vi "PathPlanner_Cmd_Follow_Internal_InitEvents.vi"(8 "TrigerEvents":bool, 9 "Reset In":bool, 11 "TrajectoryEventCommands":T5) -> (3 "UntriggeredEvents":T1[](array[typedef]))   [LabVIEW 2019, in "PathPlanner24.lvlib"]
doc: "This is an internal function. It is not to be called by end users."
uses:
  PathPlanner24.lvlib
  ENum/PathPlanner_TrajectoryEvent_Type_ENUM.ctl
  TypeDef/PathPlannerCommandUtil.ctl
  TypeDef/PathPlannerTrajectoryEvent.ctl
  ENum/PathPlanner_CommandUtil_Type_ENUM.ctl
  TypeDef/PathPlannerTrajectoryEvents.ctl
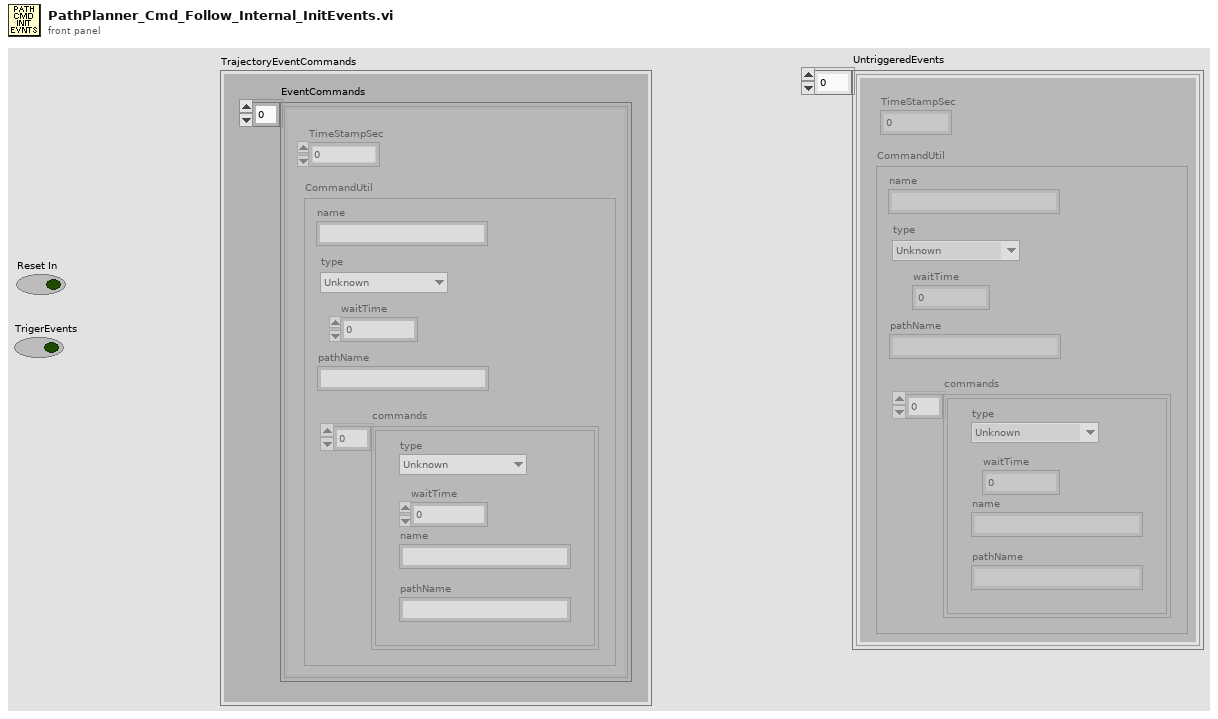
[diagram p1: front panel]
types:
  T1 = typedef "PathPlanner24.lvlib/PathPlannerTrajectoryEvent.ctl" = cluster{"TimeStampSec":dbl, "CommandUtil":T2}
  T2 = typedef "PathPlanner24.lvlib/PathPlannerCommandUtil.ctl" = cluster{"waitTime":dbl, "name":string, "pathName":string, "commands":cluster{"type":T3, "waitTime":dbl, "name":string, "pathName":string}[], "type":T4}
  T3 = typedef "PathPlanner24.lvlib/PathPlanner_TrajectoryEvent_Type_ENUM.ctl" = enum16{"Unknown", "Wait", "Named", "Path", "Sequential", "Parallel", "Race", "Deadline", "PointTowardsZoneEnter", "PointTowardsZoneExit", "TriggerEventStart", "TriggerEventStop", "TriggerEventOneshot"}
  T4 = typedef "PathPlanner24.lvlib/PathPlanner_CommandUtil_Type_ENUM.ctl" = enum16{"Unknown", "Wait", "Named", "Path", "Sequential", "Parallel", "Race", "Deadline"}
  T5 = typedef "PathPlanner24.lvlib/PathPlannerTrajectoryEvents.ctl" = cluster{"EventCommands":T1[]}
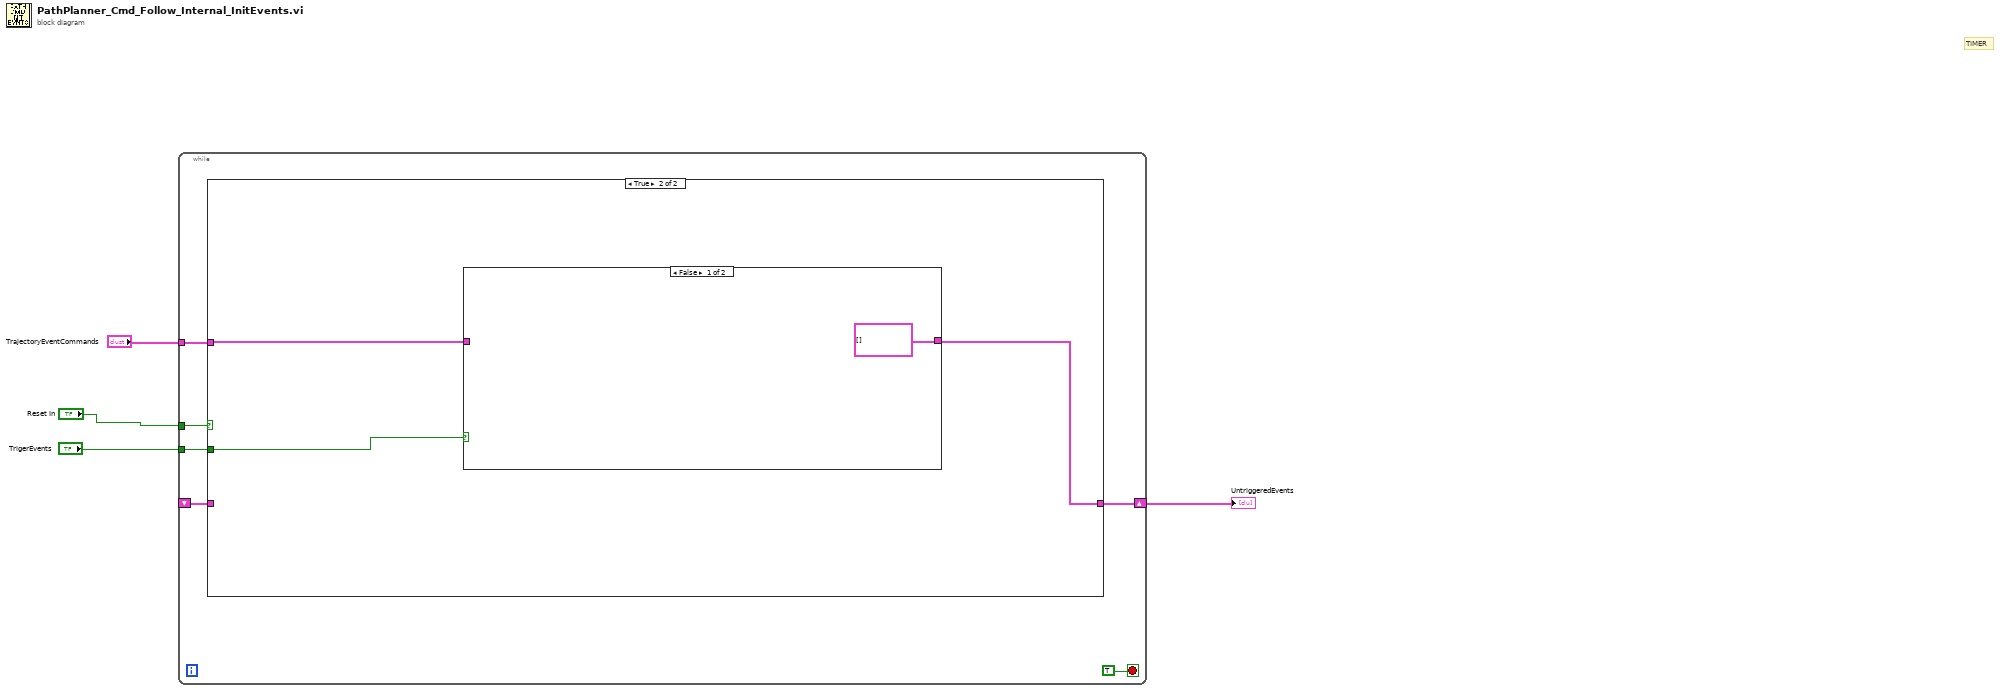
[diagram p0: block diagram]
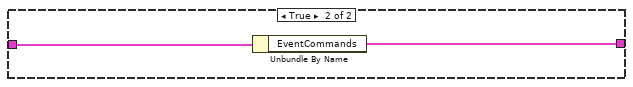
[diagram p3: hidden frame]
diagram:
  # "TIMER"
  n1 = while {
    tunnel: "TrajectoryEventCommands" -> [w10]
    tunnel: "Reset In" -> [w9]
    shift-right: [w8] -> w3
    shift-left: _ -> [w6]
    tunnel: "TrigerEvents" -> [w5]
    stop <- TRUE stop-if-true
    n2 = case shown="True" w9 {
      tunnel: w10 -> [_ w14]
      tunnel: [w11 w13] -> w8
      tunnel: w6 -> [w11 _]
      tunnel: w5 -> [_ w12]
      frame False {
      }
      frame True {
        n3 = case shown="False" w12 {
          tunnel: w14 -> [_ w17]
          tunnel: [T1[] [] ("EventCommands") w16] -> w13
          frame False {
          }
          frame True {
            n4 = Unbundle By Name(w17) -> ("EventCommands"=w16:T1[])
          }
        }
      }
    }
  }
  "UntriggeredEvents" <- w3
